vi "PicoScope2000Open.vi"(9 "error in (no error)":errorcluster) -> (1 "Unit Info":T1, 2 "handle":i16, 3 "error out":errorcluster)   [LabVIEW 2009]
doc: "This VI opens a PicoScope 3000a/b and returns a handle to the device."
uses:
  ps2000.dll
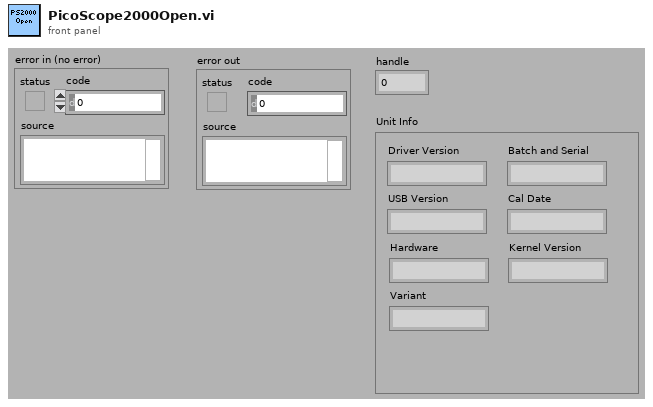
[diagram p1: front panel]
types:
  T1 = cluster{"Driver Version":string, "USB Version":string, "Hardware":string, "Variant":string, "Batch and Serial":string, "Cal Date":string, "Kernel Version":string}
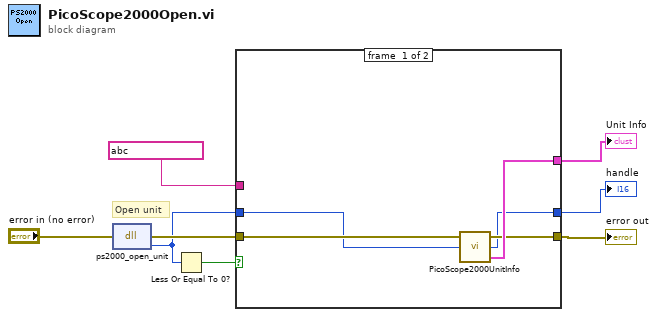
[diagram p0: block diagram]
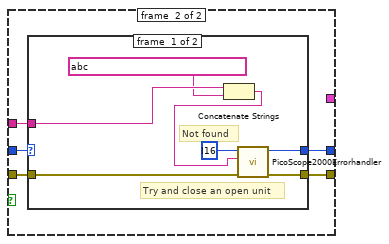
[diagram p2: hidden frame]
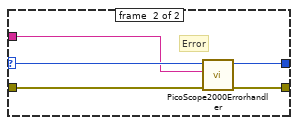
[diagram p3: hidden frame]
diagram:
  # "Open unit"
  n1 = dll-call lib="PS2000.dll" fn="ps2000_open_unit"(error in="error in (no error)") -> (error out=w7:errorcluster, "handle"=w3:i16)  [unwired: 2 in, 1 out]
  n2 = Less Or Equal To 0?(x=w3) -> (x <= 0?=w4:bool)
  n3 = case shown="True" w4 {
    tunnel: w3 -> [w10 w18]
    tunnel: [w9 w14] -> w1
    tunnel: [w11 w17] -> w5
    tunnel: w7 -> [w12 w16]
    tunnel: [w13 _] -> w6
    tunnel: string ? ("API function") -> [_ w15]
    frame #0 {
      n4 = call "PicoScope2000UnitInfo.vi"("handle in"=w10, "error in (no error)"=w12) -> ("Unit Info"=w13:T1, "handle out"=w9:i16, "error out"=w11:errorcluster)  [unwired: 1 in]
    }
    frame #1 {
      n5 = case shown="-1, Default" w18 {
        selector: w18 -> [_ w30]
        tunnel: [w25 w29] -> w14
        tunnel: [w23 w28] -> w17
        tunnel: w16 -> [w24 w27]
        tunnel: w15 -> [w20 w26]
        frame #0 {
          # "Try and close an open unit"
          # "Not found"
          n6 = Concatenate Strings(w20, string ? ("string")) -> (w21:string)
          n7 = call "PicoScope2000Errorhandler.vi"("Handle in"=i16 ?, "API function"=w21, "error in (no error)"=w24) -> ("Handle out"=w25:i16, "error out"=w23:errorcluster)  [unwired: 6 in]
        }
        frame #1 {
          # "Error"
          n8 = call "PicoScope2000Errorhandler.vi"("Handle in"=w30, "API function"=w26, "error in (no error)"=w27) -> ("Handle out"=w29:i16, "error out"=w28:errorcluster)  [unwired: 6 in]
        }
      }
    }
  }
  "handle" <- w1
  "error out" <- w5
  "Unit Info" <- w6
